vi "CO reference Mast.vi"(8 "error in (no error)":errorcluster caption="에러 입력(에러 없음)", 11 "Instrument Manager 입력":refnum<class "Instrument Manager.lvclass">) -> (0 "error out":errorcluster caption="에러 출력", 3 "Instrument Manager 출력":refnum<class "Instrument Manager.lvclass">)   [LabVIEW 2023, in "Instrument Manager.lvclass"]
uses:
  Instrument Manager.lvclass
  Module/Turn Table and Mast Control/Class/CO3000/CO3000.lvclass
  Module/Turn Table and Mast Control/Interface Class/Mast/Interface - Mast.lvclass
  Instrument Manager.lvclass/Instrument Manager.ctl
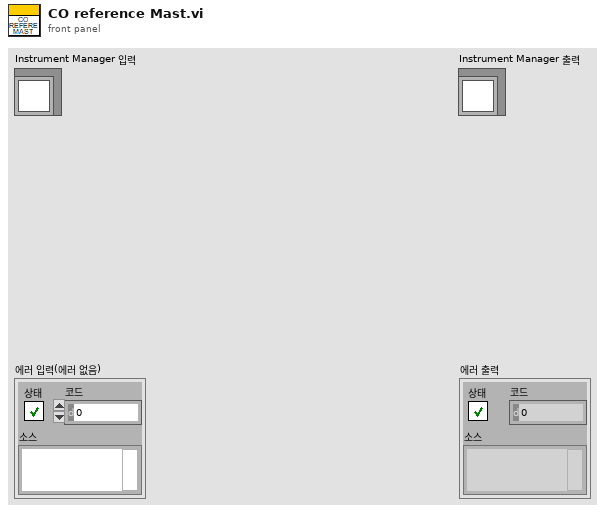
[diagram p1: front panel]
types:
  T1 = cluster{"Anritsu Call Box":refnum<class "Anritsu Call Box.lvclass">, "Spectrum Analyzer":refnum<class "Interface_Spectrum.lvclass">, "RF Switch Box":refnum<class "RF Filter Box.lvclass">, "Turn Table":refnum<class "Interface - Turn Table.lvclass">, "Mast":refnum<class "Interface - Mast.lvclass">, "3D Controller":refnum<class "Interface_3D Controller.lvclass">}
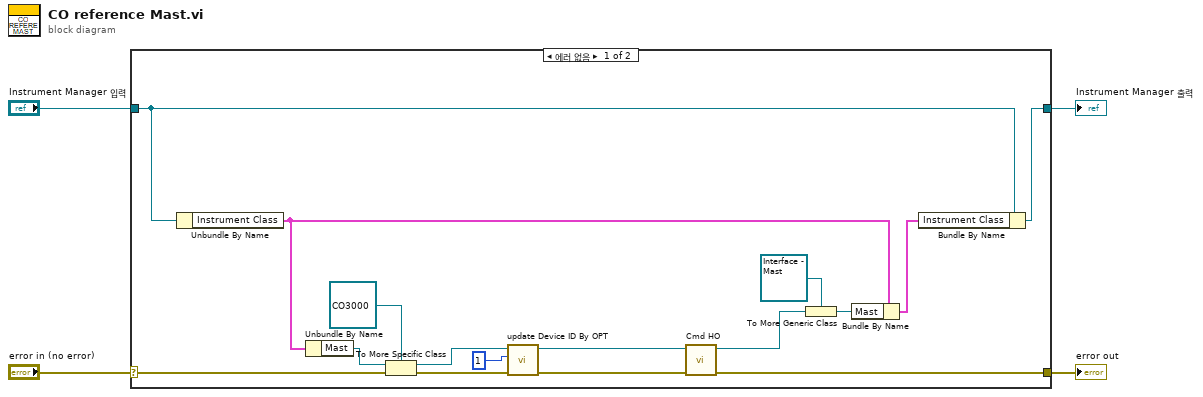
[diagram p0: block diagram]
diagram:
  n1 = case shown="에러 없음" "error in (no error)" {
    selector: "error in (no error)" -> [w18 w22]
    tunnel: [w16 w22] -> w3
    tunnel: [w13 w21] -> w1
    tunnel: "Instrument Manager 입력" -> [w15 w21]
    frame No Error {
      n2 = Unbundle By Name(w15) -> ("Instrument Class"=w17:T1)
      n3 = Unbundle By Name(w17) -> ("Mast"=w19:refnum<class "Interface - Mast.lvclass">)
      n4 = To More Specific Class(target class=refnum<class "CO3000.lvclass"> refnum ("Turn Table and Mast.lvlib:CO3000.lvclass"), reference=w19, error in=w18) -> (specific class reference=w7:refnum<class "CO3000.lvclass">, error out=w9:errorcluster)
      n5 = call "update Device ID By OPT.vi"("error in (no error)"=w9, "Mast Index"=1, "CO3000 in"=w7) -> ("error out"=w8:errorcluster, "CO3000 out"=w5:refnum<class "CO3000.lvclass">)  [unwired: 5 in, 2 out]
      n6 = call-dynamic "Cmd HO.vi"("error in (no error)"=w8, "CO3000 입력"=w5) -> ("error out"=w16:errorcluster, "CO3000 출력"=w12:refnum<class "CO3000.lvclass">)  [unwired: 8 in]
      n7 = To More Generic Class(target class=refnum<class "Interface - Mast.lvclass"> refnum ("Turn Table and Mast.lvlib:Interface - Mast.lvclass"), reference=w12) -> (generic class reference=w10:refnum<class "Interface - Mast.lvclass">)
      n8 = Bundle By Name(cluster=w17, "Mast"=w10) -> (w14:T1)
      n9 = Bundle By Name(cluster=w15, "Instrument Class"=w14) -> (w13:refnum<class "Instrument Manager.lvclass">)
    }
    frame Error {
    }
  }
  "error out" <- w3
  "Instrument Manager 출력" <- w1
